vi "LTE set BW and DL Channel.vi"(8 "error in (no error)":errorcluster caption="에러 입력(에러 없음)", 9 "PCC Downlink":i32, 10 "BandWidth":T1, 11 "Instrument Manager 입력":refnum<class "Instrument Manager.lvclass">) -> (0 "error out":errorcluster caption="에러 출력", 3 "Instrument Manager 출력":refnum<class "Instrument Manager.lvclass">)   [LabVIEW 2023, in "Instrument Manager.lvclass"]
uses:
  Instrument Manager.lvclass
  Instrument Manager.lvclass/Instrument Manager.ctl
  Module/ANRITSU Call Box/Interface Class/Anritsu Call Box.lvclass
  Module/ANRITSU Call Box/Type Definition/LTE Supported BandWidth.ctl
  Module/ANRITSU Call Box/ANRITSU Call Box.lvlib
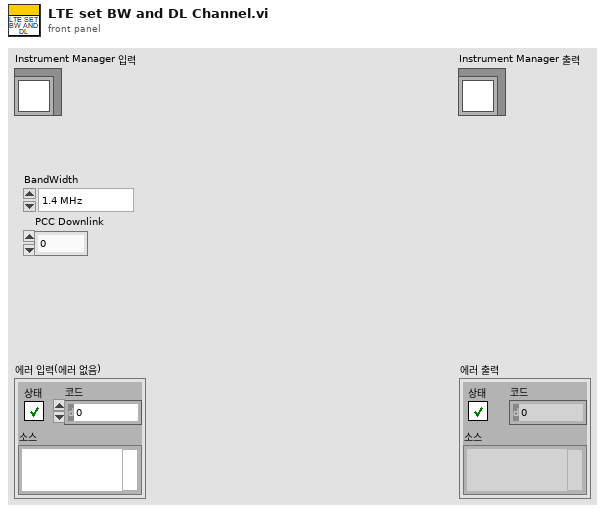
[diagram p1: front panel]
types:
  T1 = typedef "ANRITSU Call Box.lvlib/LTE Supported BandWidth.ctl" = enum16{"1.4 MHz", "3 MHz", "5 MHz", "10 MHz", "15 MHz", "20 MHz"}
  T2 = cluster{"Anritsu Call Box":refnum<class "Anritsu Call Box.lvclass">, "Spectrum Analyzer":refnum<class "Interface_Spectrum.lvclass">, "RF Switch Box":refnum<class "RF Filter Box.lvclass">, "Turn Table":refnum<class "Interface - Turn Table.lvclass">, "Mast":refnum<class "Interface - Mast.lvclass">, "3D Controller":refnum<class "Interface_3D Controller.lvclass">}
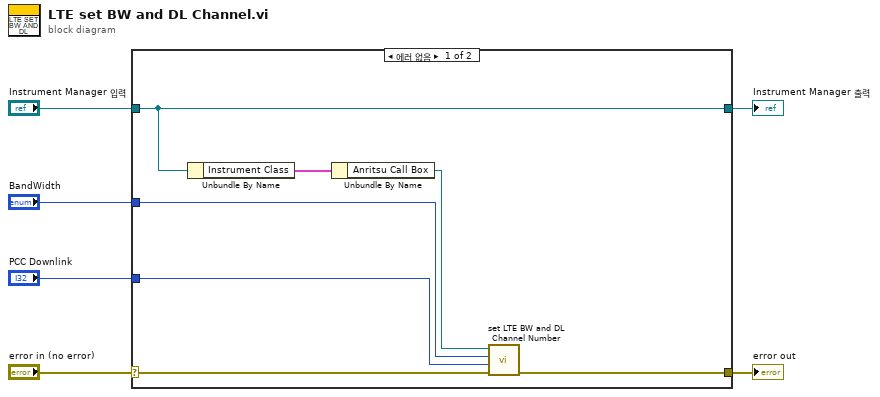
[diagram p0: block diagram]
diagram:
  n1 = case shown="에러 없음" "error in (no error)" {
    selector: "error in (no error)" -> [w13 w15]
    tunnel: [w12 w15] -> w5
    tunnel: [w11 w14] -> w3
    tunnel: "Instrument Manager 입력" -> [w11 w14]
    tunnel: "BandWidth" -> [w8 _]
    tunnel: "PCC Downlink" -> [w7 _]
    frame No Error {
      n2 = Unbundle By Name(w11) -> ("Instrument Class"=w10:T2)
      n3 = Unbundle By Name(w10) -> ("Anritsu Call Box"=w9:refnum<class "Anritsu Call Box.lvclass">)
      n4 = call-dynamic "set LTE BW and DL Channel Number.vi"("error in (no error)"=w13, "PCC Downlink"=w7, "BandWidth"=w8, "Anritsu Call Box 입력"=w9) -> ("error out"=w12:errorcluster)  [unwired: 6 in, 1 out]
    }
    frame Error {
    }
  }
  "error out" <- w5
  "Instrument Manager 출력" <- w3
